vi "Own20261012_GetNumericRepresentation.vi"() -> ()   [LabVIEW 2024]
uses:
  <vilib>/numeric/LVNumericRepresentation.ctl
panel:
  out "representation":T1 caption="表示法"
  out "error out":errorcluster caption="错误输出"
  in  "numeric_id":u32
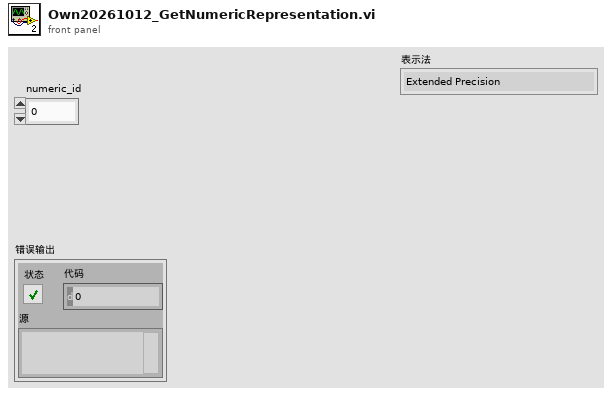
[diagram p1: front panel]
types:
  T1 = typedef "LVNumericRepresentation.ctl" = enum32{"Extended Precision", "Double Precision", "Single Precision", "Long", "Word", "Byte", "Unsigned Long", "Unsigned Word", "Unsigned Byte", "Complex Extended", "Complex Double", "Complex Single", "Quad", "Unsigned Quad", "Fixed-Point"}
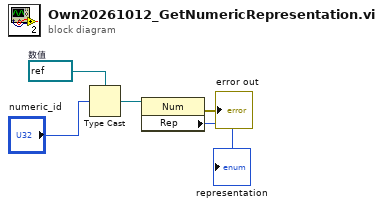
[diagram p0: block diagram]
diagram:
  w4 = refnum<vi> refnum  # 数值
  n1 = Type Cast ("强制类型转换")(type=w4, x="numeric_id") -> (*(type *) &x=w3:refnum<vi>)
  n2 = property on="属性节点" class="Num"(reference=w3) -> (error out=→"error out":errorcluster, "Rep"=→"representation":T1)  [unwired: 1 in, 1 out]
